vi "Array Extra Probe.vi"() -> ()   [LabVIEW 2026]
doc: "Round6 Task3 extra array node coverage: Replace Array Subset, Array Max & Min, Reverse 1D Array, Split Array (Split Array terminal names are a guess - undocumented in reference). Expected: Replaced=[10,5,99,3,20], MaxVal=20, MaxIdx=4, MinVal=3, MinIdx=3, Reversed=[20,3,8,5,10], SplitFront=[10,5], SplitRest=[8,3,20]."
panel:
  out "Reversed":i32[](array[numeric])
  out "MinIdx":i32
  out "MinVal":i32
  out "MaxIdx":i32
  out "MaxVal":i32
  out "Replaced":i32[](array[numeric])
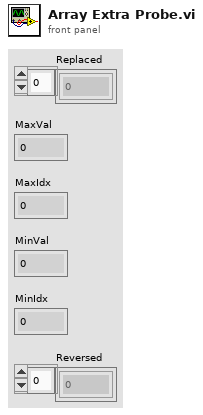
[diagram p1: front panel]
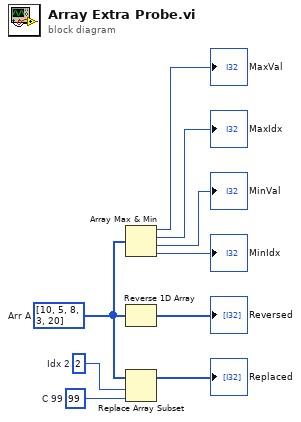
[diagram p0: block diagram]
diagram:
  w8 = 99  # C 99
  w9 = 2  # Idx 2
  w7 = i32[] [10, 5, 8, 3, 20]  # Arr A
  n1 = Array Max & Min(array=w7) -> (max value=→"MaxVal":i32, max index (indices)=→"MaxIdx":i32, min value=→"MinVal":i32, min index (indices)=→"MinIdx":i32)
  n2 = Reverse 1D Array(array=w7) -> (reversed array=→"Reversed":i32[])
  n3 = Replace Array Subset(array=w7, new element=w8, index=w9) -> (→"Replaced":i32[])
